vi "Open Transport.vi"(8 "error in":errorcluster, 11 "transport config":T3) -> (0 "error out":errorcluster, 3 "transport session":T2)   [LabVIEW 2015, in "Lengmur_socket.lvlib"]
uses:
  Lengmur_socket.lvlib
  Types/Transport Config.ctl
  Types/Transport Kind.ctl
  <vilib>/Instr/_visa.llb/VISA Configure Serial Port (Instr).vi
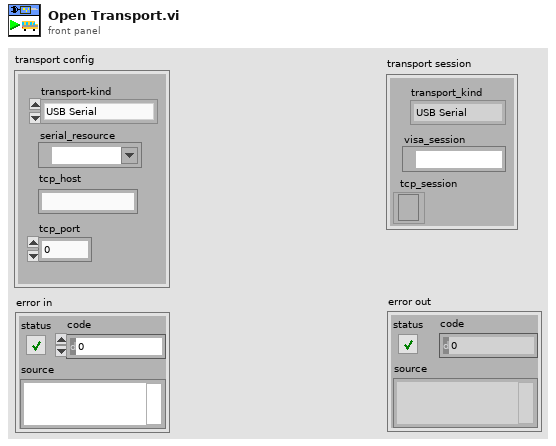
[diagram p1: front panel]
types:
  T1 = typedef "Lengmur_socket.lvlib/Transport Kind.ctl" = enum16{"USB Serial", "Ethernet TCP"}
  T2 = cluster{"transport_kind":T1, "visa_session":refnum<visa-resource-name>, "tcp_session":refnum<k5>}
  T3 = typedef "Lengmur_socket.lvlib/Transport Config.ctl" = cluster{"transport-kind":T1, "serial_resource":refnum<visa-resource-name>, "tcp_host":string, "tcp_port":u16}
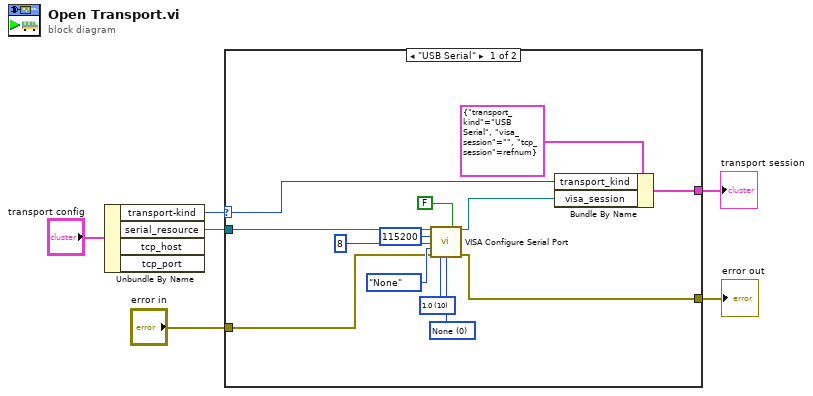
[diagram p0: block diagram]
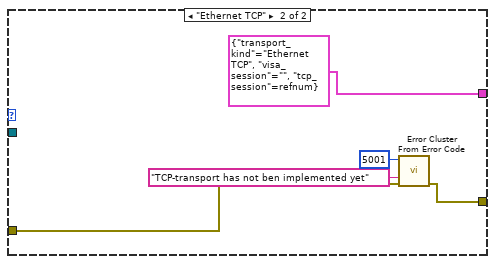
[diagram p2: hidden frame]
diagram:
  n1 = Unbundle By Name("transport config") -> ("transport-kind"=w6:T1, "serial_resource"=w5:refnum<visa-resource-name>)  [unwired: 2 out]
  n2 = case shown="\"USB Serial\"" w6 {
    selector: w6 -> [w9 _]
    tunnel: w5 -> [w19 _]
    tunnel: "error in" -> [w12 w24]
    tunnel: [w11 w21] -> w3
    tunnel: [w7 T2 {"transport_kind"=enum."Ethernet TCP", "visa_session"="", "tcp_session"=refnum} ("transport_session")] -> w2
    frame "USB Serial" {
      w14 = u16 0 items=["None", "XON/XOFF", "RTS/CTS", "XON/XOFF & RTS/CTS", "DTR/DSR", "XON/XOFF & DTR/DSR"] ("flow control (0:none)")
      w17 = u16 10 items=["1.0"=10, "1.5"=15, "2.0"=20] ("stop bits (10: 1 bit)")
      n3 = call-poly "VISA Configure Serial Port"("VISA resource name"=w19, "Enable Termination\nChar (T)"=FALSE ("Enable Termination\nChar (T)"), "baud rate (9600)"=u32 115200, "data bits (8)"=u16 8, "parity (0:none)"=enum16{"None", "Odd", "Even", "Mark", "Space"}."None", "error in (no error)"=w12, "stop bits (10: 1 bit)"=w17, "flow control (0:none)"=w14) -> ("VISA resource name out"=w8:refnum<visa-resource-name>, "error out"=w11:errorcluster)  [unwired: 6 in]
      n4 = Bundle By Name(cluster=T2 {"transport_kind"=enum."USB Serial", "visa_session"="", "tcp_session"=refnum} ("transport_session"), "transport_kind"=w9, "visa_session"=w8) -> (w7:T2)
    }
    frame "Ethernet TCP" {
      n5 = call <vilib>:"Error Cluster From Error Code.vi"("error in (no error)"=w24, "error message (\"\")"="TCP-transport has not ben implemented yet" ("error message (\"\")"), "error code (0)"=5001) -> ("error out"=w21:errorcluster)  [unwired: 6 in]
    }
  }
  "transport session" <- w2
  "error out" <- w3
